vi "Toast With Images.vi"() -> ()   [LabVIEW 2020]
doc: "Shows a Windows toast with a hero image using ToastBuilder. The included PNG illustrates a simulated battery discharge. See Detailed Help for the expected rendering and image path requirements."
uses:
  ToastNotification/Activation.ctl
  ToastNotification/Argument.ctl
  PlugIns/UserEventActivationHandler/UserEventActivationHandler.lvclass
  C:/Users/loicw/Documents/LabVIEW/ToastNotifications/Sources/ActivationHandler/ActivationHandler.lvclass
  PlugIns/UserEventActivationHandler/UserEventActivationHandler.lvclass/UserEventActivationHandler.ctl
  PlugIns/UserEventActivationHandler/Read Event Ref.vi
  ToastBuilder/ToastBuilder.lvclass
  C:/Users/loicw/Documents/LabVIEW/ToastNotifications/Sources/ToastSource/ToastSource.lvclass
  ToastBuilder/Create ToastBuilder.vi
  ToastService/ToastService.lvclass
  ToastNotification/ToastNotification.lvlib
panel:
  out "error out":errorcluster
  out "Toast XML":string
  in  "error in":errorcluster
  out "Activation":T1
  out "error":errorcluster
  in  "stop":bool
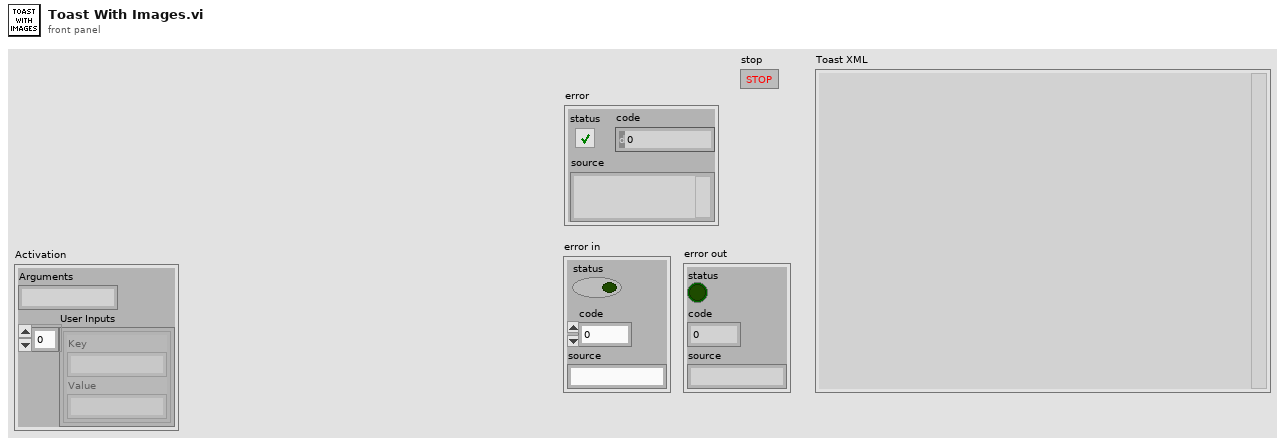
[diagram p1: front panel]
types:
  T1 = typedef "ToastNotification.lvlib/Activation.ctl" = cluster{"Arguments":string, "User Inputs":T2[]}
  T2 = typedef "ToastNotification.lvlib/Argument.ctl" = cluster{"Key":string, "Value":string}
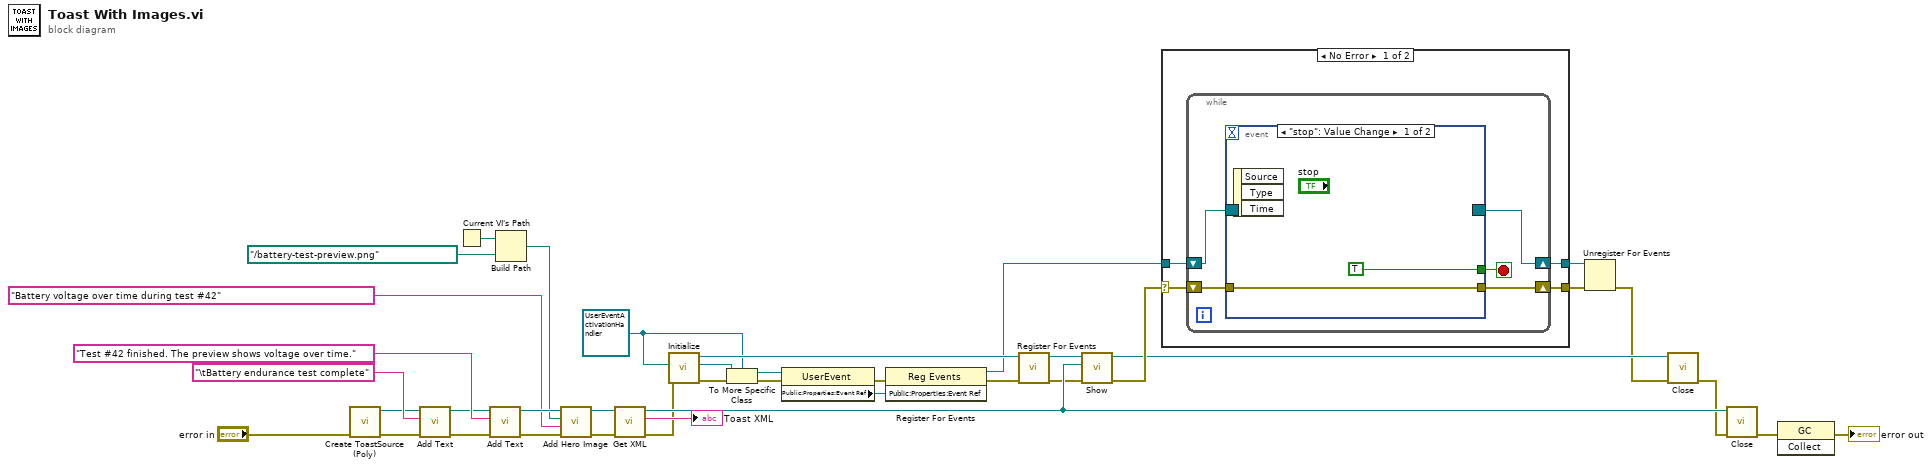
[diagram p0: block diagram]
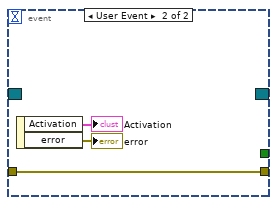
[diagram p2: hidden frame]
diagram:
  w20 = refnum<class "UserEventActivationHandler.lvclass"> refnum
  n1 = call-poly "Create ToastSource (Poly).vi"("error in"="error in") -> ("error out"=w33:errorcluster, "ToastBuilder out"=w32:refnum<class "ToastBuilder.lvclass">)  [unwired: 9 in]
  n2 = call "Add Text.vi"("error in"=w33, "text"="\tBattery endurance test complete", "ToastBuilder in"=w32) -> ("error out"=w36:errorcluster, "ToastBuilder out"=w35:refnum<class "ToastBuilder.lvclass">)  [unwired: 7 in]
  n3 = Current VI's Path() -> (path=w3:path)
  n4 = call "Add Text.vi"("error in"=w36, "text"="Test #42 finished. The preview shows voltage over time.", "ToastBuilder in"=w35) -> ("error out"=w7:errorcluster, "ToastBuilder out"=w8:refnum<class "ToastBuilder.lvclass">)  [unwired: 7 in]
  n5 = Build Path(base path=w3, name or relative path=path "../battery-test-preview.png" ("Image")) -> (appended path=w1:path)
  n6 = call "Add Hero Image.vi"("error in (no error)"=w7, "alternateText"="Battery voltage over time during test #42", "Image"=w1, "ToastBuilder in"=w8) -> ("error out"=w5:errorcluster, "ToastBuilder out"=w6:refnum<class "ToastBuilder.lvclass">)  [unwired: 6 in]
  n7 = call-dynamic "Get XML.vi"("error in"=w5, "ToastBuilder in"=w6) -> ("error out"=w29:errorcluster, "GetContent"=→"Toast XML":string, "ToastBuilder out"=w30:refnum<class "ToastBuilder.lvclass">)  [unwired: 7 in]
  n8 = call "Initialize.vi"("error in (no error)"=w29, "ActivationHandler in"=w20) -> ("error out"=w27:errorcluster, "ActivationHandler out"=w19:refnum<class "UserEventActivationHandler.lvclass">, "ToastService out"=w26:refnum<class "ToastService.lvclass">)  [unwired: 7 in]
  n9 = To More Specific Class(target class=w20, reference=w19, error in=w27) -> (specific class reference=w17:refnum<class "UserEventActivationHandler.lvclass">, error out=w21:errorcluster)
  n10 = property class="UserEvent"(reference=w17, error in=w21) -> (error out=w18:errorcluster, "Public:Properties:Event Ref"=w15:refnum<user-event>)  [unwired: 1 out]
  n11 = register-events(error in=w18, w15) -> (reference out=w11:refnum<event-registration>, error out=w16:errorcluster)  [unwired: 1 in]
  n12 = call "Register For Events.vi"("error in (no error)"=w16, "ToastService in"=w26) -> ("error out"=w10:errorcluster, "ToastService out"=w9:refnum<class "ToastService.lvclass">)  [unwired: 8 in]
  n13 = call "Show.vi"("error in (no error)"=w10, "ToastSource in"=w30, "ToastService in"=w9) -> ("error out"=w25:errorcluster, "ToastService out"=w24:refnum<class "ToastService.lvclass">)  [unwired: 7 in]
  n14 = case shown="No Error" w25 {
    selector: w25 -> [w42 w53]
    tunnel: [w41 w53] -> w14
    tunnel: w11 -> [w40 w54]
    tunnel: [w39 w54] -> w12
    frame No Error {
      n15 = while {
        shift-right: [w46] -> w41
        shift-left: w42 -> [w47]
        shift-right: [w44] -> w39
        shift-left: w40 -> [w45]
        stop <- w43 stop-if-true
        n16 = event shown="[0] \"stop\": Value Change" {
          selector: w45 -> [_ _]
          dyn-events: [_ _] -> w44
          timeout: _ -> [_ _]
          tunnel: [w49 w52] -> w46
          tunnel: w47 -> [w49 w52]
          tunnel: [TRUE _] -> w43
          event "stop": Value Change {
            n17 = event-data() -> ()  [unwired: 1 in, 3 out]
          }
          event User Event {
            n18 = event-data() -> ("Activation"=→"Activation":T1, "error"=→"error":errorcluster)  [unwired: 1 in]
          }
        }
      }
    }
    frame Error {
    }
  }
  n19 = Unregister For Events(event registration refnum=w12, error in=w14) -> (error out=w13:errorcluster)
  n20 = call "Close.vi"("error in (no error)"=w13, "ToastService in"=w24) -> ("error out"=w28:errorcluster)  [unwired: 9 in]
  n21 = call-dynamic "Close.vi"("error in"=w28, "ToastBuilder in"=w30) -> ("error out"=w23:errorcluster)  [unwired: 9 in]
  n22 = invoke class="GC" method="Collect"(error in=w23) -> (error out=→"error out":errorcluster)  [unwired: 2 in, 2 out]
